vi "FuncVI_Sub - VI - Open VI Reference (Name or Path as String).vi"(8 "error in":errorcluster, 9 "options":i32, 10 "VI name or path":string) -> (0 "error out":errorcluster, 3 "VI Refnum":refnum<vi>)   [LabVIEW 2021]
doc: "::: CalcExpress Toolkit :::\nCopyright (c) 2000-2026 Konstantin Shifershteyn. All rights reserved."
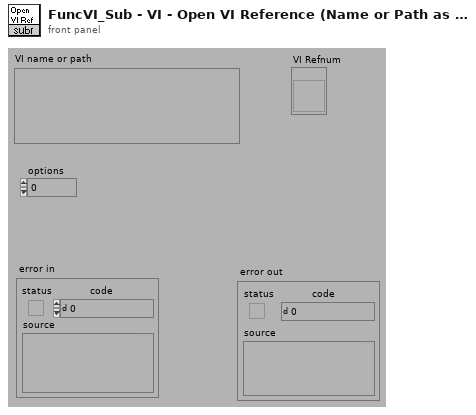
[diagram p1: front panel]
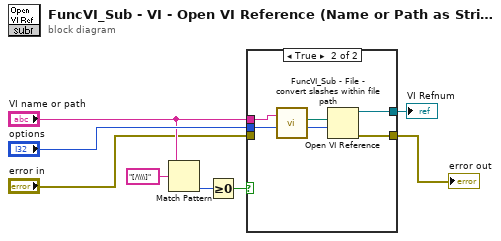
[diagram p0: block diagram]
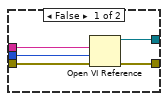
[diagram p2: hidden frame]
diagram:
  n1 = Match Pattern(string="VI name or path", regular expression="[/\\\\]") -> (offset past match=w7:i32)  [unwired: 1 in, 3 out]
  n2 = Greater Or Equal To 0?(x=w7) -> (x >= 0?=w4:bool)
  n3 = case shown="True" w4 {
    tunnel: "options" -> [w13 w18]
    tunnel: "VI name or path" -> [w12 w16]
    tunnel: [w11 w15] -> w3
    tunnel: [w10 w14] -> w2
    tunnel: "error in" -> [w9 _]
    frame False {
      n4 = Open VI Reference(vi path=w12, options=w13, error in (no error)=w9) -> (vi reference=w11:refnum<vi>, error out=w10:errorcluster)  [unwired: 3 in]
    }
    frame True {
      n5 = call "FuncVI_Sub - File - convert slashes within file path.vi"("str: path"=w16) -> ("path out"=w17:path)  [unwired: 3 in, 1 out]
      n6 = Open VI Reference(vi path=w17, options=w18) -> (vi reference=w15:refnum<vi>, error out=w14:errorcluster)  [unwired: 4 in]
    }
  }
  "error out" <- w2
  "VI Refnum" <- w3
